vi "Val Tinit.vi"(1 "Port COM run 1 REG":refnum<visa-resource-name> caption="Port RS232", 2 "Adresse":u8, 3 "Onglet_Tinit":enum32{"Définir Tinit", "Acquérir Tinit"}(ring), 4 "Val T ini":dbl=20.0) -> (0 "Température":dbl)   [LabVIEW 2022 SP3]
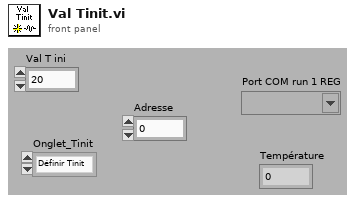
[diagram p1: front panel]
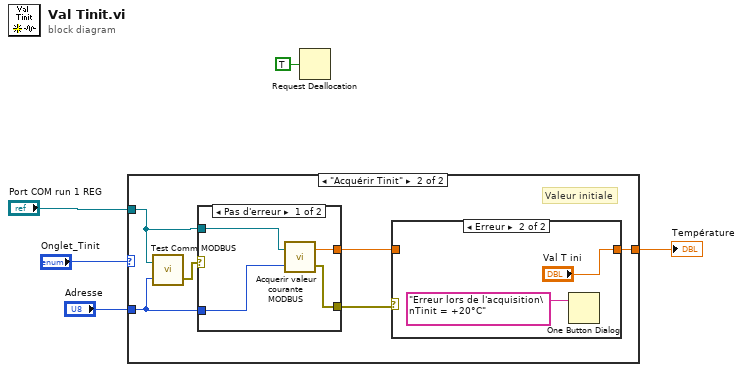
[diagram p0: block diagram]
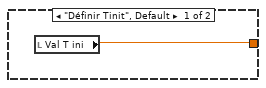
[diagram p2: hidden frame]
diagram:
  n1 = case shown="\"Acquérir Tinit\"" "Onglet_Tinit" {
    tunnel: [w6 w8] -> w2
    tunnel: "Adresse" -> [_ w10]
    tunnel: "Port COM run 1 REG" -> [_ w9]
    frame "Définir Tinit", Default {
      n2 = local read "Val T ini"() -> (w6:dbl)
    }
    frame "Acquérir Tinit" {
      # "Valeur initiale"
      n3 = call "Test Comm MODBUS.vi"("Adresse rég"=w10, "Port COM run 1 REG"=w9) -> ("error out"=w12:errorcluster)  [unwired: 1 in]
      n4 = case shown="Pas d'erreur" w12 {
        selector: w12 -> [_ w17]
        tunnel: [w16 _] -> w7
        tunnel: w10 -> [w15 _]
        tunnel: [w14 w17] -> w11
        tunnel: w9 -> [w13 _]
        frame No Error {
          n5 = call "Acquerir valeur courante MODBUS.vi"("Adresse régulateur"=w15, "Port COM run 1 REG"=w13) -> ("sortie d'erreur"=w14:errorcluster, "Température"=w16:dbl)
        }
        frame Error {
        }
      }
      n6 = case shown="Erreur" w11 {
        tunnel: [w18 "Val T ini"] -> w8
        tunnel: w7 -> [w18 _]
        frame No Error {
        }
        frame Error {
          n7 = One Button Dialog(message="Erreur lors de l'acquisition\nTinit = +20°C") -> ()  [unwired: 1 in, 1 out]
        }
      }
    }
  }
  "Température" <- w2
  n8 = Request Deallocation(TRUE ("flag")) -> ()
